vi "Test données alarmes.vi"() -> (1 "Booléen":bool)   [LabVIEW 2022 SP3]
uses:
  Variables globales/Variables glob EUROTHERM.vi
panel:
  out "Dernieres donnees regs":cluster{"Dernieres donnees 1COM":string[][]}[](array[cluster])
  # "VRAI = donnée AL est vide ou\nn'est pas un chiffre\nexemple : \"TO\", \"dialogue ...\""
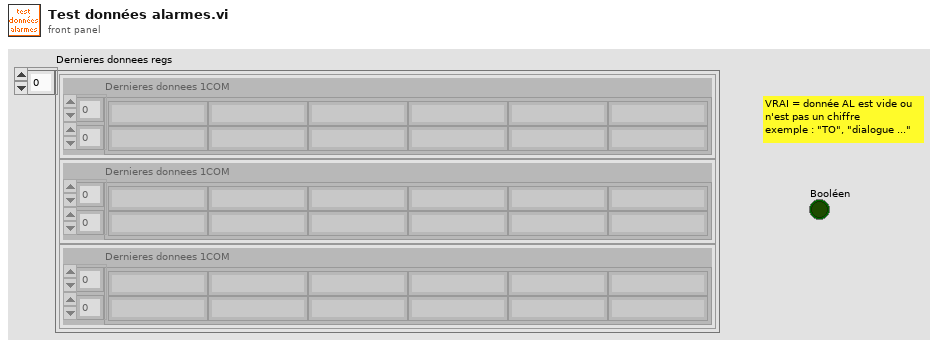
[diagram p1: front panel]
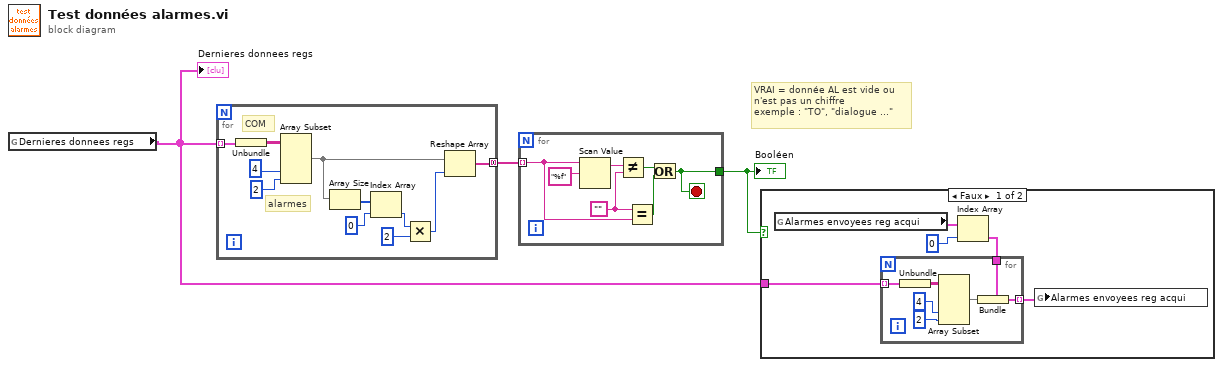
[diagram p0: block diagram]
diagram:
  # "VRAI = donnée AL est vide ou\nn'est pas un chiffre\nexemple : \"TO\", \"dialogue ...\""
  n1 = global read "Variables glob EUROTHERM.vi" "Dernieres donnees regs"() -> (w1:cluster{"Dernieres donnees 1COM":string[][]}[])
  "Dernieres donnees regs" <- w1
  n2 = for {
    tunnel: w1 -> [w14] mode=indexing
    tunnel: [w10] -> w3 mode=concatenating
    # "COM"
    # "alarmes"
    n3 = Unbundle(w14) -> ("Dernieres donnees 1COM"=w11:string[][])
    n4 = Array Subset(array=w11, index (col)=4 ("indice"), length (col)=2 ("longueur")) -> (w9:string[][])  [unwired: 2 in]
    n5 = Array Size(array=w9) -> (size(s)=w8:i32[])
    n6 = Index Array(array=w8, index=0 ("indice")) -> (element=w6:i32)
    n7 = Multiply(x=w6, y=2) -> (x*y=w4:i32)
    n8 = Reshape Array(w9, w4) -> (w10:string[])
  }
  n9 = for {
    tunnel: w3 -> [w16] mode=indexing
    tunnel: [w15] -> w2
    stop <- w15 stop-if-true
    w21 = ""
    n10 = Scan Value(string=w16, format string="%f" ("chaîne de format")) -> (output string=w18:string)  [unwired: 1 in, 1 out]
    n11 = Not Equal?(x=w18, y=w21) -> (x != y?=w19:bool)
    n12 = Equal?(x=w21, y=w16) -> (x = y?=w20:bool)
    n13 = Or(x=w19, y=w20) -> (x .or. y?=w15:bool)
  }
  "Booléen" <- w2
  n14 = case shown="Faux" w2 {
    tunnel: w1 -> [w26 _]
    frame False {
      n15 = global read "Variables glob EUROTHERM.vi" "Alarmes envoyees reg acqui"() -> (w24:cluster{"alarmes 1COM reg":string[][]}[])
      n16 = Index Array(array=w24, index=0 ("indice")) -> (element=w22:cluster{"alarmes 1COM reg":string[][]})
      n17 = for {
        tunnel: w26 -> [w33] mode=indexing
        tunnel: w22 -> [w29]
        tunnel: [w27] -> w25 mode=indexing
        n18 = Unbundle(w33) -> ("Dernieres donnees 1COM"=w32:string[][])
        n19 = Array Subset(array=w32, index (col)=4 ("indice"), length (col)=2 ("longueur")) -> (w28:string[][])  [unwired: 2 in]
        n20 = Bundle(cluster=w29, "alarmes 1COM reg"=w28) -> (w27:cluster{"alarmes 1COM reg":string[][]})
      }
      n21 = global write "Variables glob EUROTHERM.vi" "Alarmes envoyees reg acqui"(w25) -> ()
    }
    frame True {
    }
  }
